vi "ControllerElapsedTime.vi"(10 "TimeNow":dbl, 11 "InData":T1) -> (3 "Elapsed":dbl)   [LabVIEW 2026]
uses:
  Controls/DataType.ctl
  Controls/StateType.ctl
  Controls/ModeType.ctl
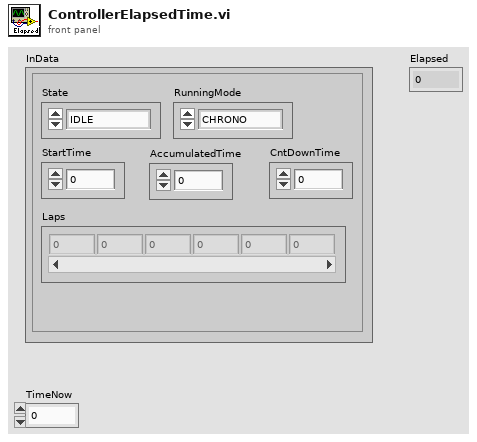
[diagram p1: front panel]
types:
  T1 = typedef "DataType.ctl" = cluster{"State":T2, "RunningMode":T3, "StartTime":dbl, "AccumulatedTime":dbl, "CntDownTime":dbl, "Laps":dbl[]}
  T2 = typedef "StateType.ctl" = enum16{"IDLE", "RUNNING", "PAUSED", "FINISHED"}
  T3 = typedef "ModeType.ctl" = enum16{"CHRONO", "COUNTDOWN", ""}
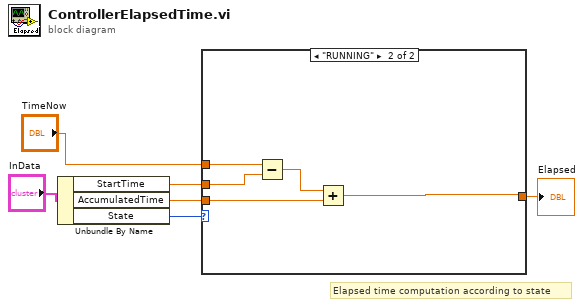
[diagram p0: block diagram]
diagram:
  # "Elapsed time computation according to state"
  n1 = Unbundle By Name("InData") -> ("StartTime"=w3:dbl, "AccumulatedTime"=w4:dbl, "State"=w5:T2)
  n2 = case shown="\"RUNNING\"" w5 {
    tunnel: w4 -> [w7 w11]
    tunnel: w3 -> [_ w10]
    tunnel: "TimeNow" -> [_ w9]
    tunnel: [w7 w8] -> w1
    frame "IDLE", "PAUSED", "FINISHED" {
    }
    frame "RUNNING" {
      n3 = Subtract(x=w9, y=w10) -> (x-y=w12:dbl)
      n4 = Add(x=w12, y=w11) -> (x+y=w8:dbl)
    }
  }
  "Elapsed" <- w1
